vi "Get Paths.vi"(8 "error in (no error)":errorcluster, 11 "ParseXML in":refnum<class "ParseSVG.lvclass">) -> (0 "error out":errorcluster, 3 "ParseXML out":refnum<class "ParseSVG.lvclass">)   [LabVIEW 2019, in "ParseSVG.lvclass"]
uses:
  ParseSVG.lvclass
  Path.ctl
  ParseSVG.lvclass/ParseSVG.ctl
  Read RawXML.vi
  <userlib>/_OpenG.lib/lvdata/lvdata.llb/Get Data Name__ogtk.vi
  <userlib>/_OpenG.lib/lvdata/lvdata.llb/Get Cluster Element Names__ogtk.vi
  <userlib>/_OpenG.lib/lvdata/lvdata.llb/Array of VData to VCluster__ogtk.vi
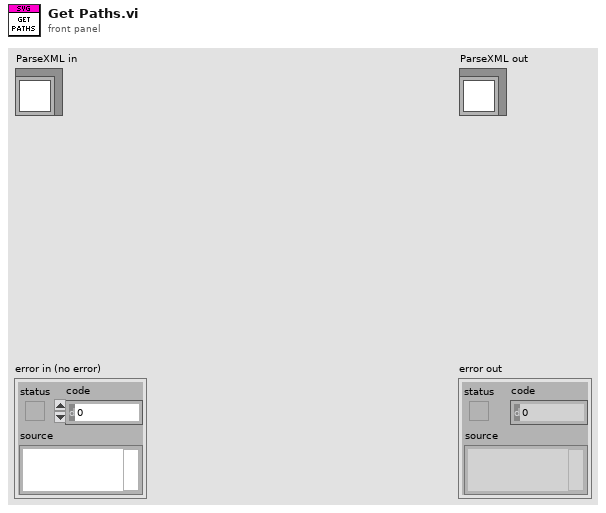
[diagram p1: front panel]
types:
  T1 = typedef "ParseSVG.lvclass/Path.ctl" = cluster{"d":string, "style":string, "transform":string, "id":string}
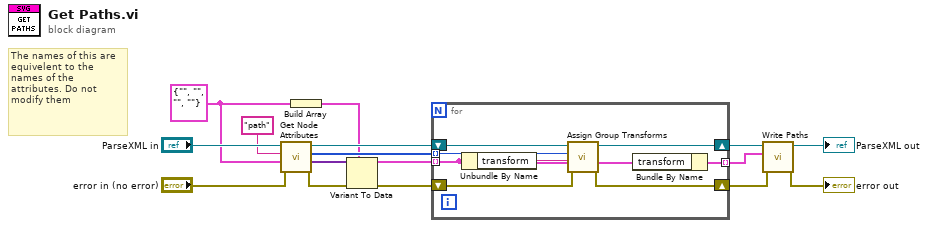
[diagram p0: block diagram]
diagram:
  w9 = T1 {"d"="", "style"="", "transform"="", "id"=""} ("Path")
  # "The names of this are equivelent to the names of the attributes. Do not modify them"
  n1 = call "Get Node Attributes.vi"("error in (no error)"="error in (no error)", "Attributes Cluster"=w9, "Node Name (exact)"="path", "ParseSVG in"="ParseXML in") -> ("error out"=w12:errorcluster, "[Attributes Cluster]"=w13:variant[], "Positions"=w3:i32[], "ParseSVG out"=w8:refnum<class "ParseSVG.lvclass">)  [unwired: 4 in]
  n2 = Build Array(w9) -> (w1:T1[])
  n3 = Variant To Data(error in=w12, type=w1, Variant=w13) -> (data=w4:T1[], error out=w6:errorcluster)
  n4 = for {
    shift-right: [w24] -> w7
    shift-left: w8 -> [w25]
    shift-right: [w22] -> w5
    shift-left: w6 -> [w23]
    tunnel: w4 -> [w19] mode=indexing
    tunnel: w3 -> [w20] mode=indexing
    tunnel: [w17] -> w2 mode=indexing
    n5 = Unbundle By Name(w19) -> ("transform"=w21:string)
    n6 = call "Assign Group Transforms.vi"("error in (no error)"=w23, "transform in"=w21, "position"=w20, "ParseSVG in"=w25) -> ("error out"=w22:errorcluster, "transform out"=w18:string, "ParseSVG out"=w24:refnum<class "ParseSVG.lvclass">)  [unwired: 5 in]
    n7 = Bundle By Name(cluster=w19, "transform"=w18) -> (w17:T1)
  }
  n8 = call "Write Paths.vi"("error in (no error)"=w5, "Paths"=w2, "ParseXML in"=w7) -> ("error out"=→"error out":errorcluster, "ParseXML out"=→"ParseXML out":refnum<class "ParseSVG.lvclass">)  [unwired: 7 in]
